vi "PicoScope5000aAdvancedTriggerSettingsV2.vi"(0 "error in":errorcluster, 1 "handle in":i16=16384, 3 "Trigger Conditions":T1 {"Digital Port 1" items=["Don't Care", "True", "False"]; "Digital Port 0" items=["Don't Care", "True", "False"]; "PWQ" items=["Don't Care", "True", "False"]; "Aux" items=["Don't Care", "True", "False"]; "Ext" items=["Don't Care", "True", "False"]; "Channel D" items=["Don't Care", "True", "False"]; "Channel C" items=["Don't Care", "True", "False"]; "Channel B" items=["Don't Care", "True", "False"]; "Channel A" items=["Don't Care", "True", "False"]; "Condition Logic" items=["AND", "OR", "XOR"]}, 4 "Trigger Delay":u32, 5 "Auto Trigger (us)":u64=1000000, 6 "Channel A Trigger Properties":T4={"thresholdUpper"=0, "thresholdUpperHysteresis"=0, "thresholdLower"=0, "thresholdLowerHysteresis"=0, "Threshold Mode"=0, "Direction"=2, "Available"=FALSE} {"Direction" items=["Above / Inside", "Below / Outside", "Rising / Enter", "Falling / Exit", "Rising or Falling / Enter or Exit", "Above Lower", "Below Lower", "Rising Lower", "Falling Lower", "Positive Runt", "Negative Runt"]; "Threshold Mode" items=["Level", "Window"]}, 7 "Channel D Trigger Properties":T4={"thresholdUpper"=0, "thresholdUpperHysteresis"=0, "thresholdLower"=0, "thresholdLowerHysteresis"=0, "Threshold Mode"=0, "Direction"=2, "Available"=FALSE} {"Direction" items=["Above / Inside", "Below / Outside", "Rising / Enter", "Falling / Exit", "Rising or Falling / Enter or Exit", "Above Lower", "Below Lower", "Rising Lower", "Falling Lower", "Positive Runt", "Negative Runt"]; "Threshold Mode" items=["Level", "Window"]}, 8 "Channel B Trigger Properties":T4={"thresholdUpper"=0, "thresholdUpperHysteresis"=0, "thresholdLower"=0, "thresholdLowerHysteresis"=0, "Threshold Mode"=0, "Direction"=2, "Available"=FALSE} {"Direction" items=["Above / Inside", "Below / Outside", "Rising / Enter", "Falling / Exit", "Rising or Falling / Enter or Exit", "Above Lower", "Below Lower", "Rising Lower", "Falling Lower", "Positive Runt", "Negative Runt"]; "Threshold Mode" items=["Level", "Window"]}, 10 "Digital Port  0":T3 {"Direction Channel 7" items=["Don't Care", "Low", "High", "Rising", "Falling"]; "Direction Channel 6" items=["Don't Care", "Low", "High", "Rising", "Falling"]; "Direction Channel 5" items=["Don't Care", "Low", "High", "Rising", "Falling"]; "Direction Channel 4" items=["Don't Care", "Low", "High", "Rising", "Falling"]; "Direction Channel 3" items=["Don't Care", "Low", "High", "Rising", "Falling"]; "Direction Channel 2" items=["Don't Care", "Low", "High", "Rising", "Falling"]; "Direction Channel 1" items=["Don't Care", "Low", "High", "Rising", "Falling"]; "Direction Channel 0" items=["Don't Care", "Low", "High", "Rising", "Falling"]}, 11 "Ext. Trigger Properties":T4={"thresholdUpper"=0, "thresholdUpperHysteresis"=0, "thresholdLower"=0, "thresholdLowerHysteresis"=0, "Threshold Mode"=0, "Direction"=2, "Available"=FALSE} {"Direction" items=["Above / Inside", "Below / Outside", "Rising / Enter", "Falling / Exit", "Rising or Falling / Enter or Exit", "Above Lower", "Below Lower", "Rising Lower", "Falling Lower", "Positive Runt", "Negative Runt"]; "Threshold Mode" items=["Level", "Window"]}, 12 "Digital Port  1":T2 {"Direction Channel 15" items=["Don't Care", "Low", "High", "Rising", "Falling"]; "Direction Channel 14" items=["Don't Care", "Low", "High", "Rising", "Falling"]; "Direction Channel 13" items=["Don't Care", "Low", "High", "Rising", "Falling"]; "Direction Channel 12" items=["Don't Care", "Low", "High", "Rising", "Falling"]; "Direction Channel 11" items=["Don't Care", "Low", "High", "Rising", "Falling"]; "Direction Channel 10" items=["Don't Care", "Low", "High", "Rising", "Falling"]; "Direction Channel 9" items=["Don't Care", "Low", "High", "Rising", "Falling"]; "Direction Channel 8" items=["Don't Care", "Low", "High", "Rising", "Falling"]}, 13 "Aux. Trigger Properties (DO NOT USE)":T4={"thresholdUpper"=0, "thresholdUpperHysteresis"=0, "thresholdLower"=0, "thresholdLowerHysteresis"=0, "Threshold Mode"=0, "Direction"=2, "Available"=FALSE} {"Direction" items=["Above / Inside", "Below / Outside", "Rising / Enter", "Falling / Exit", "Rising or Falling / Enter or Exit", "Above Lower", "Below Lower", "Rising Lower", "Falling Lower", "Positive Runt", "Negative Runt"]; "Threshold Mode" items=["Level", "Window"]}, 16 "Channel C Trigger Properties":T4={"thresholdUpper"=0, "thresholdUpperHysteresis"=0, "thresholdLower"=0, "thresholdLowerHysteresis"=0, "Threshold Mode"=0, "Direction"=2, "Available"=FALSE} {"Direction" items=["Above / Inside", "Below / Outside", "Rising / Enter", "Falling / Exit", "Rising or Falling / Enter or Exit", "Above Lower", "Below Lower", "Rising Lower", "Falling Lower", "Positive Runt", "Negative Runt"]; "Threshold Mode" items=["Level", "Window"]}, 18 "Pulse Width Qualifier Conditions":T6 {"Condition Logic" items=["AND", "OR", "XOR"]}, 19 "Pulse Width Qualifier Settings":T5={"Direction"=2, "Lower Limit"=0, "Upper Limit"=0, "Pulse Width Type"=0} {"Pulse Width Type" items=["None", "Less Than", "Greater Than", "In Range", "Out of Range"]; "Direction" items=["Rising"=2, "Falling"=3, "Rising Lower"=7, "Above"=0, "Below"=1, "Rising or Falling"=4, "Falling Lower"=8, "Below Lower"=6, "Above Lower"=5]}) -> (14 "error out":errorcluster, 15 "handle out":i16=16384)   [LabVIEW 2010]
doc: "This VI is an interface for the advanced trigger features of the oscilloscope (Using V2 functions now recommended)\nA simple trigger can be set using PicoScope5000aSettings.vi, in which case it is not necessary to use this VI."
uses:
  ps5000a.dll
panel:
  out "XOR Debug Array":u32[][](array[numeric])
  in  "SetTrigger Info Action XOR":bool=TRUE
  in  "SetTrigger Info Action OR":bool=TRUE
  # "For Condition Logic Suggested settings;\nFor AND, XOR logic-(parallel triggers)\nUse level-type triggers (Level or Inside/outside Window Triggers)\n\nFor OR logic- (single channel)\nUse edge types (e.g. rising, falling, entering window)"
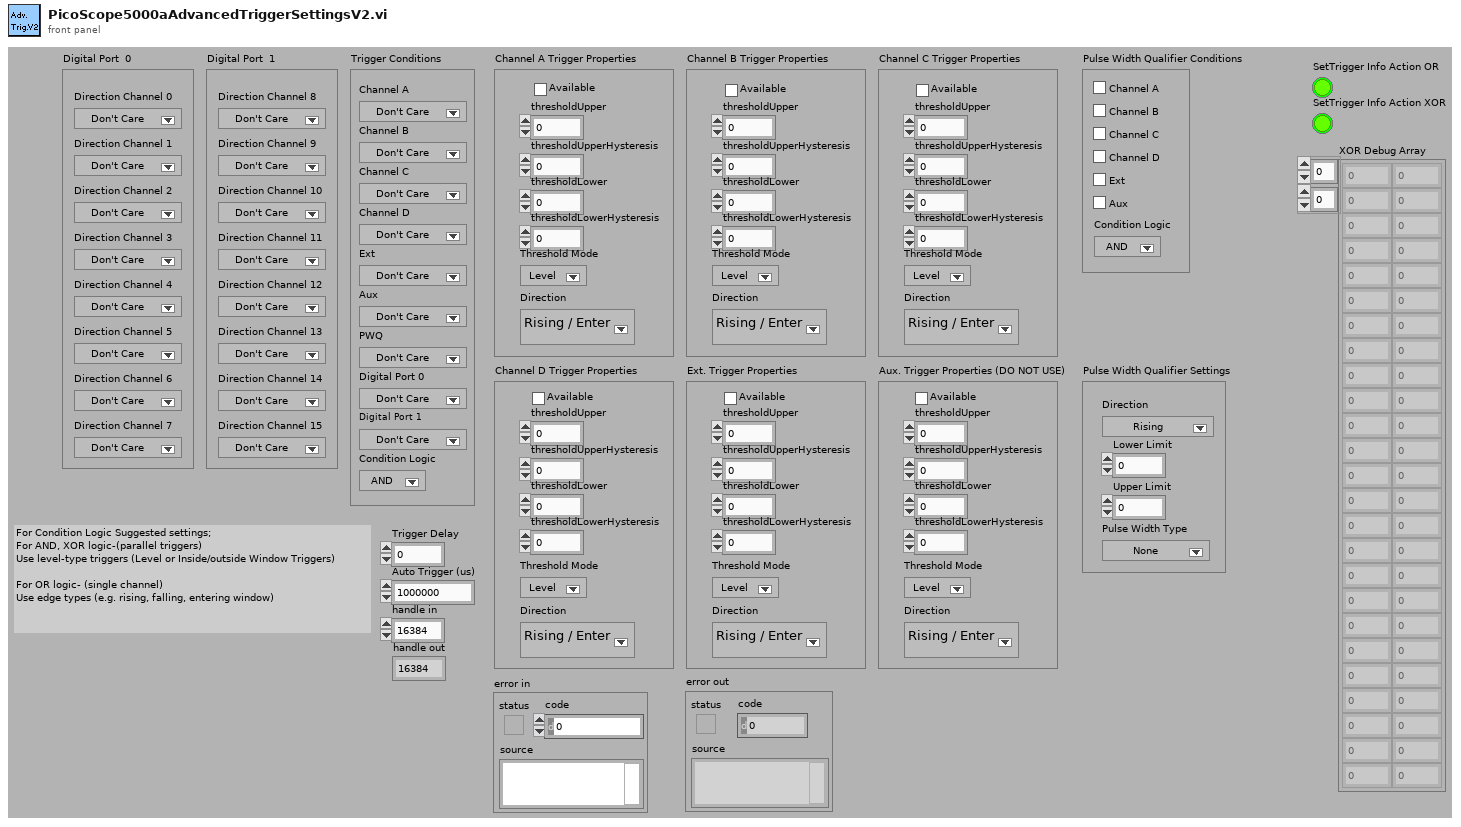
[diagram p1: front panel]
types:
  T1 = cluster{"Channel A":u16, "Channel B":u16, "Channel C":u16, "Channel D":u16, "Ext":u16, "Aux":u16, "PWQ":u16, "Digital Port 0":u16, "Digital Port 1":u16, "Condition Logic":u16}
  T2 = cluster{"Direction Channel 8":u16, "Direction Channel 9":u16, "Direction Channel 10":u16, "Direction Channel 11":u16, "Direction Channel 12":u16, "Direction Channel 13":u16, "Direction Channel 14":u16, "Direction Channel 15":u16}
  T3 = cluster{"Direction Channel 0":u16, "Direction Channel 1":u16, "Direction Channel 2":u16, "Direction Channel 3":u16, "Direction Channel 4":u16, "Direction Channel 5":u16, "Direction Channel 6":u16, "Direction Channel 7":u16}
  T4 = cluster{"thresholdUpper":i16, "thresholdUpperHysteresis":u16, "thresholdLower":i16, "thresholdLowerHysteresis":u16, "Threshold Mode":i32, "Direction":i32, "Available":bool}
  T5 = cluster{"Direction":u32, "Lower Limit":u32, "Upper Limit":u32, "Pulse Width Type":u32}
  T6 = cluster{"Channel A":bool, "Channel B":bool, "Channel C":bool, "Channel D":bool, "Aux":bool, "Condition Logic":u16, "Ext":bool}
  T7 = cluster{"thresholdUpper":i16, "thresholdUpperHysteresis":u16, "thresholdLower":i16, "thresholdLowerHysteresis":u16, "Threshold Mode":i32, "Direction":i32, "Available":bool}[]
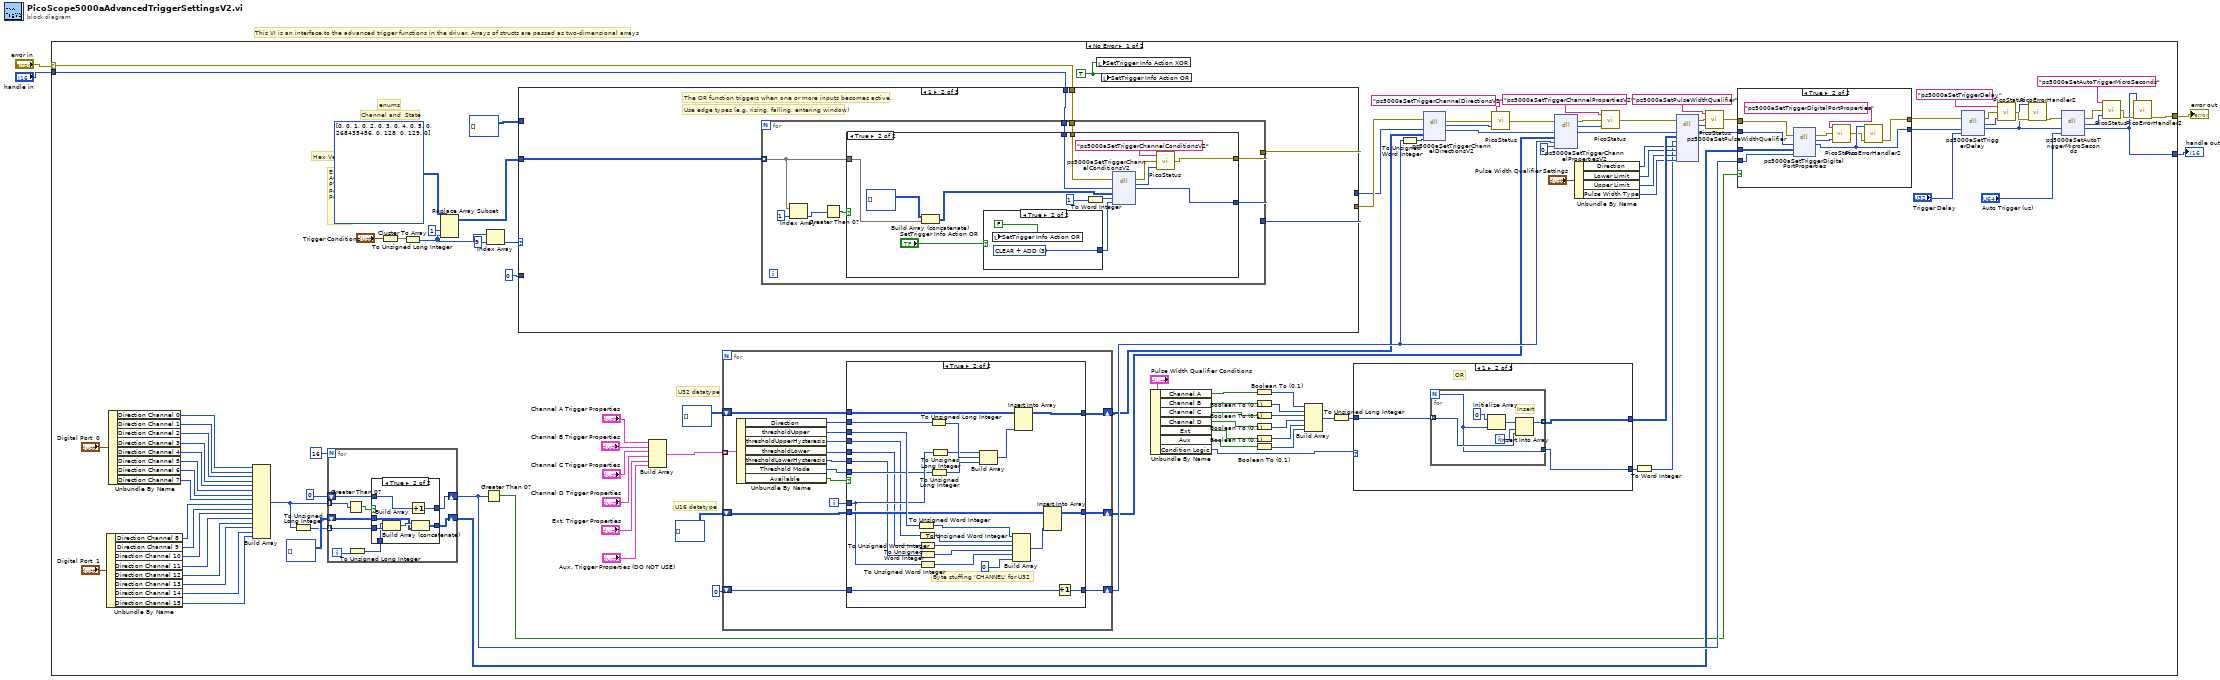
[diagram p0: block diagram]
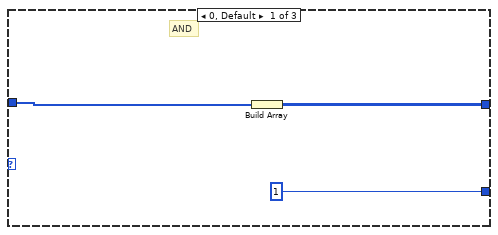
[diagram p4: hidden frame]
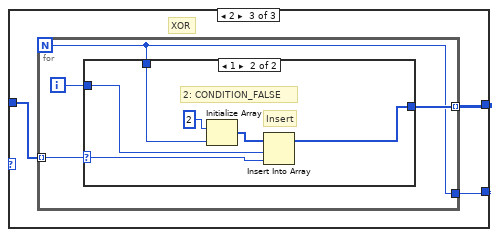
[diagram p5: hidden frame]
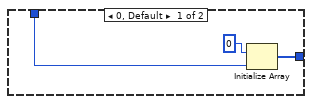
[diagram p6: hidden frame]
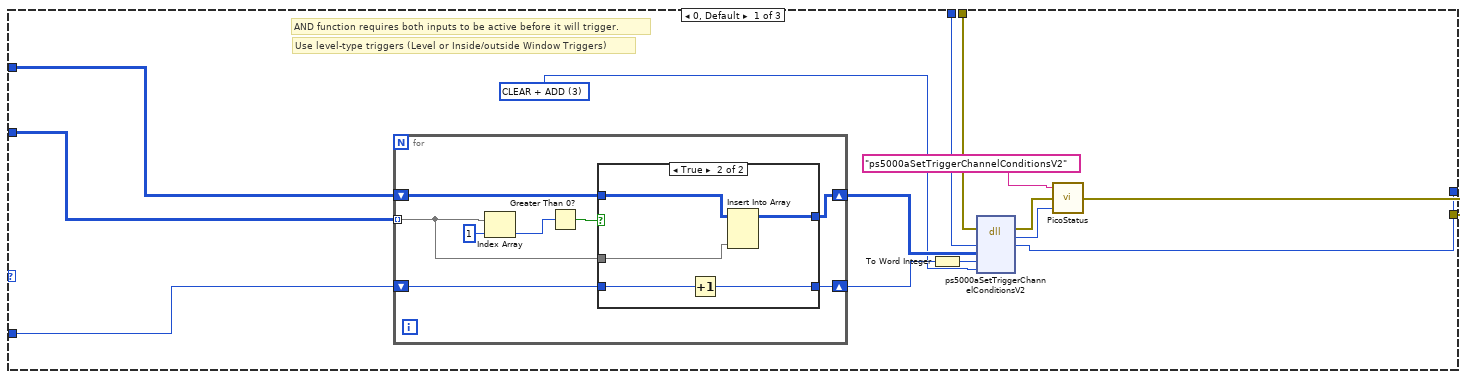
[diagram p8: hidden frame]
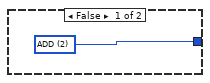
[diagram p11: hidden frame]
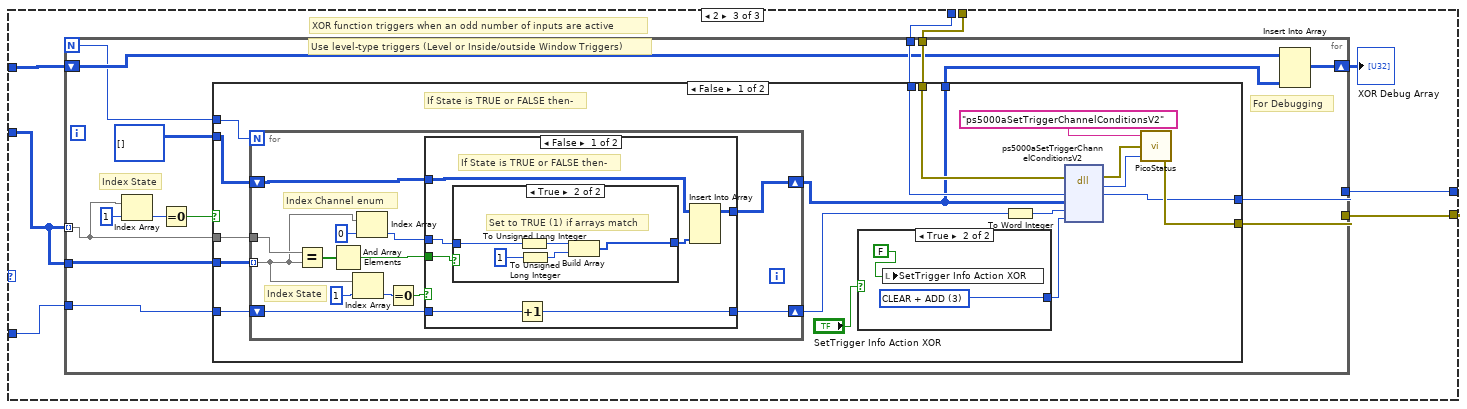
[diagram p12: hidden frame]
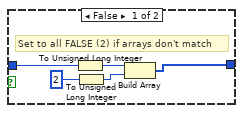
[diagram p13: hidden frame]
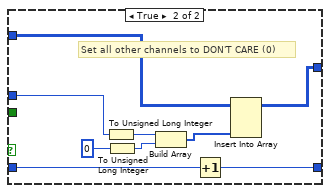
[diagram p14: hidden frame]
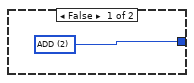
[diagram p15: hidden frame]
diagram:
  # "This VI is an interface to the advanced trigger functions in the driver. Arrays of structs are passed as two-dimensional arrays"
  n1 = case shown="No Error" "error in" {
    selector: "error in" -> [w46 w362]
    tunnel: "handle in" -> [w45 w363]
    tunnel: [w33 w363] -> w2
    tunnel: [w34 w362] -> w1
    frame No Error {
      w39 = TRUE ("Boolean")
      # "enums"
      # "Ext\nAux\nPWQ\nPort0\nPort1"
      # "Channel and  State"
      # "Hex Values"
      # "U16 datatype"
      # "U32 datatype"
      n2 = Unbundle By Name("Digital Port  1") -> ("Direction Channel 8"=w71:u16, "Direction Channel 9"=w70:u16, "Direction Channel 10"=w69:u16, "Direction Channel 11"=w68:u16, "Direction Channel 12"=w67:u16, "Direction Channel 13"=w66:u16, "Direction Channel 14"=w65:u16, "Direction Channel 15"=w64:u16)
      n3 = Unbundle By Name("Digital Port  0") -> ("Direction Channel 0"=w63:u16, "Direction Channel 1"=w80:u16, "Direction Channel 2"=w79:u16, "Direction Channel 3"=w78:u16, "Direction Channel 4"=w77:u16, "Direction Channel 5"=w76:u16, "Direction Channel 6"=w75:u16, "Direction Channel 7"=w74:u16)
      n4 = Build Array(w63, w80, w79, w78, w77, w76, w75, w74, w71, w70, w69, w68, w67, w66, w65, w64) -> (w52:u16[])
      n5 = To Unsigned Long Integer(number=w52) -> (unsigned 32bit integer=w53:u32[])
      n6 = for {
        N: 16 -> [_]
        tunnel: w53 -> [w134] mode=indexing
        shift-right: [w135] -> w57
        shift-left: i16 0 -> [w136]
        shift-right: [w132] -> w56
        shift-left: u32[][] [] -> [w133]
        tunnel: w52 -> [w130] mode=indexing
        i -> [w129]
        n7 = Greater Than 0?(x=w130) -> (x > 0?=w131:bool)
        n8 = To Unsigned Long Integer(number=w129) -> (unsigned 32bit integer=w128:u32)
        n9 = case shown="True" w131 {
          tunnel: w136 -> [w138 w145]
          tunnel: [w138 w142] -> w135
          tunnel: w134 -> [_ w144]
          tunnel: w128 -> [_ w143]
          tunnel: w133 -> [w137 w140]
          tunnel: [w137 w139] -> w132
          frame False {
          }
          frame True {
            n10 = Build Array(w143, w144) -> (w141:u32[])
            n11 = Increment(x=w145) -> (x+1=w142:i16)
            n12 = Build Array (concatenate)(w141, w140) -> (w139:u32[][])
          }
        }
      }
      n13 = Cluster To Array(cluster="Trigger Conditions") -> (array=w28:u16[])
      n14 = To Unsigned Long Integer(number=w28) -> (unsigned 32bit integer=w26:u32[])
      n15 = Replace Array Subset(array=u32[][] [[0, 0], [1, 0], [2, 0], [3, 0], [4, 0], [5, 0], [268435456, 0], [128, 0], [129, 0]], new element=w26, index (col)=1 ("disabled index (col)")) -> (w27:u32[][])  [unwired: 1 in]
      n16 = Greater Than 0?(x=w57) -> (x > 0?=w32:bool)
      n17 = Index Array(array=w26, index=9) -> (element=w24:u32)
      n18 = case shown="1" w24 {
        tunnel: u32[][] [] -> [w229 _ w280]
        tunnel: i16 0 -> [w228 _ w277]
        tunnel: w46 -> [w222 w249 w284]
        tunnel: w45 -> [w221 w248 w283]
        tunnel: [w218 w247 w282] -> w44
        tunnel: [w217 w246 w281] -> w43
        tunnel: w27 -> [w216 w245 w278]
        frame 0, Default {
          w219 = u32 3 items=["CLEAR + ADD"=3, "CLEAR"=1, "ADD"=2] ("Condition Action")
          # "AND function requires both inputs to be active before it will trigger."
          # "Use level-type triggers (Level or Inside/outside Window Triggers)"
          n19 = for {
            shift-right: [w236] -> w224
            shift-left: w228 -> [w235]
            shift-right: [w234] -> w220
            shift-left: w229 -> [w237]
            tunnel: w216 -> [w232] mode=indexing
            n20 = Index Array(array=w232, index=1) -> (element=w231:u32)
            n21 = Greater Than 0?(x=w231) -> (x > 0?=w233:bool)
            n22 = case shown="True" w233 {
              tunnel: w237 -> [w239 w244]
              tunnel: [w239 w243] -> w234
              tunnel: [w238 w242] -> w236
              tunnel: w235 -> [w238 w241]
              tunnel: w232 -> [_ w240]
              frame False {
              }
              frame True {
                n23 = Increment(x=w241) -> (x+1=w242:i16)
                n24 = Insert Into Array(array=w244, new element=w240) -> (w243:u32[][])  [unwired: 2 in]
              }
            }
          }
          n25 = To Word Integer(number=w224) -> (16bit integer=w227:i16)
          n26 = dll-call lib="ps5000a.dll" fn="ps5000aSetTriggerChannelConditionsV2" ("ps3000.dll:_ps3000_open_unit@0")(error in=w222, "handle"=w221, "conditions"=w220, "nConditions"=w227, "info"=w219) -> (error out=w226:errorcluster, "PICO_STATUS"=w225:u32, "handle"=w217:i16)  [unwired: 5 in, 1 out]
          n27 = call "PicoStatus.vi"("PICO STATUS"=w225, "error in"=w226, "source"="ps5000aSetTriggerChannelConditionsV2") -> ("error out"=w218:errorcluster)
        }
        frame 1 {
          # "Use edge types (e.g. rising, falling, entering window)"
          # "The OR function triggers when one or more inputs becomes active."
          n28 = for {
            tunnel: w249 -> [w257]
            tunnel: w248 -> [w256]
            tunnel: [w255] -> w247
            tunnel: [w254] -> w246
            tunnel: w245 -> [w252] mode=indexing
            n29 = Index Array(array=w252, index=1) -> (element=w251:u32)
            n30 = Greater Than 0?(x=w251) -> (x > 0?=w250:bool)
            n31 = case shown="True" w250 {
              tunnel: w257 -> [w258 w269]
              tunnel: w256 -> [w259 w268]
              tunnel: [w258 w266] -> w255
              tunnel: [w259 w265] -> w254
              tunnel: w252 -> [_ w260]
              frame False {
              }
              frame True {
                n32 = Build Array (concatenate)(u32[][] [], w260) -> (w262:u32[][])
                n33 = case shown="True" "SetTrigger Info Action OR" {
                  tunnel: [w274 w276] -> w267
                  frame False {
                    w274 = u32 2 items=["CLEAR"=1, "ADD"=2, "CLEAR + ADD"=3] ("Condition Action")
                  }
                  frame True {
                    w276 = u32 3 items=["CLEAR"=1, "ADD"=2, "CLEAR + ADD"=3] ("Condition Action")
                    n34 = local write "SetTrigger Info Action OR"(FALSE ("Boolean")) -> ()
                  }
                }
                n35 = To Word Integer(number=i16 1) -> (16bit integer=w273:i16)
                n36 = dll-call lib="ps5000a.dll" fn="ps5000aSetTriggerChannelConditionsV2" ("ps3000.dll:_ps3000_open_unit@0")(error in=w269, "handle"=w268, "conditions"=w262, "nConditions"=w273, "info"=w267) -> (error out=w272:errorcluster, "PICO_STATUS"=w271:u32, "handle"=w265:i16)  [unwired: 5 in, 1 out]
                n37 = call "PicoStatus.vi"("PICO STATUS"=w271, "error in"=w272, "source"="ps5000aSetTriggerChannelConditionsV2") -> ("error out"=w266:errorcluster)
              }
            }
          }
        }
        frame 2 {
          # "Use level-type triggers (Level or Inside/outside Window Triggers)"
          # "XOR function triggers when an odd number of inputs are active"
          n38 = for {
            N -> [w292]
            tunnel: w284 -> [w299]
            tunnel: w283 -> [w298]
            tunnel: [w297] -> w282
            tunnel: [w296] -> w281
            shift-right: [w294] -> w279
            shift-left: w280 -> [w295]
            tunnel: w278 -> [w286] mode=indexing
            tunnel: w278 -> [w289]
            tunnel: w277 -> [w290]
            # "Index State"
            # "For Debugging"
            n39 = Index Array(array=w286, index=1) -> (element=w287:u32)
            n40 = Equal To 0?(x=w287) -> (x = 0?=w285:bool)
            n41 = case shown="False" w285 {
              tunnel: w299 -> [w316 w359]
              tunnel: w298 -> [w315 w360]
              tunnel: [w314 w359] -> w297
              tunnel: [w313 w360] -> w296
              tunnel: [w311 w361] -> w293
              tunnel: w292 -> [w310 _]
              tunnel: u32[][] [] -> [w309 w361]
              tunnel: w290 -> [w308 _]
              tunnel: w289 -> [w307 _]
              tunnel: w286 -> [w306 _]
              frame False {
                # "If State is TRUE or FALSE then-"
                n42 = for {
                  N: w310 -> [_]
                  shift-right: [w328] -> w312
                  shift-left: w308 -> [w329]
                  shift-right: [w317] -> w311
                  shift-left: w309 -> [w318]
                  tunnel: w306 -> [w325]
                  tunnel: w307 -> [w321] mode=indexing
                  # "Index State"
                  # "Index Channel enum"
                  n43 = Equal?(x=w325, y=w321) -> (x = y?=w319:bool[])
                  n44 = And Array Elements(Boolean array=w319) -> (logical AND=w324:bool)
                  n45 = Index Array(array=w321, index=1) -> (element=w322:u32)
                  n46 = Index Array(array=w321, index=0) -> (element=w326:u32)
                  n47 = Equal To 0?(x=w322) -> (x = 0?=w320:bool)
                  n48 = case shown="False" w320 {
                    tunnel: w329 -> [w336 w347]
                    tunnel: [w335 w348] -> w328
                    tunnel: w326 -> [w334 w351]
                    tunnel: w324 -> [w333 _]
                    tunnel: w318 -> [w332 w350]
                    tunnel: [w330 w349] -> w317
                    frame False {
                      # "If State is TRUE or FALSE then-"
                      n49 = case shown="True" w333 {
                        tunnel: [w341 w346] -> w331
                        tunnel: w334 -> [w340 w345]
                        frame False {
                          # "Set to all FALSE (2) if arrays don't match"
                          n50 = To Unsigned Long Integer(number=w340) -> (unsigned 32bit integer=w338:u32)
                          n51 = To Unsigned Long Integer(number=u32 2) -> (unsigned 32bit integer=w339:u32)
                          n52 = Build Array(w338, w339) -> (w341:u32[])
                        }
                        frame True {
                          # "Set to TRUE (1) if arrays match"
                          n53 = To Unsigned Long Integer(number=w345) -> (unsigned 32bit integer=w343:u32)
                          n54 = To Unsigned Long Integer(number=u32 1) -> (unsigned 32bit integer=w344:u32)
                          n55 = Build Array(w343, w344) -> (w346:u32[])
                        }
                      }
                      n56 = Increment(x=w336) -> (x+1=w335:i16)
                      n57 = Insert Into Array(array=w332, new element=w331) -> (w330:u32[][])  [unwired: 2 in]
                    }
                    frame True {
                      # "Set all other channels to DON'T CARE (0)"
                      n58 = To Unsigned Long Integer(number=w351) -> (unsigned 32bit integer=w353:u32)
                      n59 = To Unsigned Long Integer(number=u32 0) -> (unsigned 32bit integer=w354:u32)
                      n60 = Build Array(w353, w354) -> (w355:u32[])
                      n61 = Increment(x=w347) -> (x+1=w348:i16)
                      n62 = Insert Into Array(array=w350, new element=w355) -> (w349:u32[][])  [unwired: 2 in]
                    }
                  }
                }
                n63 = case shown="True" "SetTrigger Info Action XOR" {
                  tunnel: [w356 w358] -> w300
                  frame False {
                    w356 = u32 2 items=["CLEAR + ADD"=3, "CLEAR"=1, "ADD"=2] ("Condition Action")
                  }
                  frame True {
                    w358 = u32 3 items=["CLEAR + ADD"=3, "CLEAR"=1, "ADD"=2] ("Condition Action")
                    n64 = local write "SetTrigger Info Action XOR"(FALSE ("Boolean")) -> ()
                  }
                }
                n65 = To Word Integer(number=w312) -> (16bit integer=w305:i16)
                n66 = dll-call lib="ps5000a.dll" fn="ps5000aSetTriggerChannelConditionsV2" ("ps3000.dll:_ps3000_open_unit@0")(error in=w316, "handle"=w315, "conditions"=w311, "nConditions"=w305, "info"=w300) -> (error out=w304:errorcluster, "PICO_STATUS"=w303:u32, "handle"=w313:i16)  [unwired: 5 in, 1 out]
                n67 = call "PicoStatus.vi"("PICO STATUS"=w303, "error in"=w304, "source"="ps5000aSetTriggerChannelConditionsV2") -> ("error out"=w314:errorcluster)
              }
              frame True {
              }
            }
            n68 = Insert Into Array(array=w295, new element=w293) -> (w294:u32[][])  [unwired: 2 in]
          }
          "XOR Debug Array" <- w279
        }
      }
      n69 = Build Array("Channel A Trigger Properties", "Channel B Trigger Properties", "Channel C Trigger Properties", "Channel D Trigger Properties", "Ext. Trigger Properties", "Aux. Trigger Properties (DO NOT USE)") -> (w111:T7)
      n70 = for {
        tunnel: w111 -> [w183] mode=indexing
        shift-right: [w180] -> w49
        shift-left: i16 0 -> [w179]
        shift-right: [w177] -> w22
        shift-left: u16[][] [] -> [w178]
        shift-right: [w176] -> w23
        shift-left: u32[][] [] -> [w175]
        i -> [w181]
        n71 = Unbundle By Name(w183) -> ("Direction"=w174:i32, "thresholdUpper"=w188:i16, "thresholdUpperHysteresis"=w187:u16, "thresholdLower"=w186:i16, "thresholdLowerHysteresis"=w185:u16, "Threshold Mode"=w184:i32, "Available"=w182:bool)
        n72 = case shown="True" w182 {
          tunnel: w188 -> [_ w215]
          tunnel: w187 -> [_ w195]
          tunnel: w186 -> [_ w194]
          tunnel: w185 -> [_ w193]
          tunnel: w184 -> [_ w203]
          tunnel: w181 -> [_ w205]
          tunnel: [w191 w213] -> w180
          tunnel: w179 -> [w191 w212]
          tunnel: [w190 w210] -> w177
          tunnel: w178 -> [w190 w209]
          tunnel: [w189 w208] -> w176
          tunnel: w175 -> [w189 w207]
          tunnel: w174 -> [_ w204]
          frame False {
          }
          frame True {
            # "Byte stuffing 'CHANNEL' for U32"
            n73 = To Unsigned Word Integer(number=w215) -> (unsigned 16bit integer=w197:u16)
            n74 = To Unsigned Word Integer(number=w195) -> (unsigned 16bit integer=w196:u16)
            n75 = To Unsigned Word Integer(number=w194) -> (unsigned 16bit integer=w192:u16)
            n76 = To Unsigned Word Integer(number=w193) -> (unsigned 16bit integer=w198:u16)
            n77 = To Unsigned Word Integer(number=w205) -> (unsigned 16bit integer=w199:u16)
            n78 = To Unsigned Long Integer(number=w204) -> (unsigned 32bit integer=w201:u32)
            n79 = To Unsigned Long Integer(number=w203) -> (unsigned 32bit integer=w202:u32)
            n80 = To Unsigned Long Integer(number=w205) -> (unsigned 32bit integer=w200:u32)
            n81 = Build Array(w200, w201, w202) -> (w206:u32[])
            n82 = Build Array(w197, w196, w192, w198, w199, u16 0 ("element")) -> (w211:u16[])
            n83 = Insert Into Array(array=w207, new element=w206) -> (w208:u32[][])  [unwired: 2 in]
            n84 = Insert Into Array(array=w209, new element=w211) -> (w210:u16[][])  [unwired: 2 in]
            n85 = Increment(x=w212) -> (x+1=w213:i16)
          }
        }
      }
      n86 = local write "SetTrigger Info Action XOR"(w39) -> ()
      n87 = local write "SetTrigger Info Action OR"(w39) -> ()
      n88 = Unbundle By Name("Pulse Width Qualifier Conditions") -> ("Channel A"=w14:bool, "Channel B"=w13:bool, "Channel C"=w12:bool, "Channel D"=w11:bool, "Ext"=w10:bool, "Aux"=w9:bool, "Condition Logic"=w7:u16)
      n89 = Boolean To (0,1)(Boolean=w14) -> (0, 1=w17:i16)
      n90 = Boolean To (0,1)(Boolean=w13) -> (0, 1=w18:i16)
      n91 = Boolean To (0,1)(Boolean=w12) -> (0, 1=w19:i16)
      n92 = Boolean To (0,1)(Boolean=w11) -> (0, 1=w20:i16)
      n93 = Boolean To (0,1)(Boolean=w10) -> (0, 1=w21:i16)
      n94 = Boolean To (0,1)(Boolean=w9) -> (0, 1=w16:i16)
      n95 = Build Array(w17, w18, w19, w20, w21, w16) -> (w15:i16[])
      n96 = To Unsigned Long Integer(number=w15) -> (unsigned 32bit integer=w8:u32[])
      n97 = case shown="1" w7 {
        tunnel: [w148 w151 w160] -> w109
        tunnel: [u32 1 w149 w159] -> w6
        tunnel: w8 -> [w146 w150 w158]
        frame 0, Default {
          # "AND"
          n98 = Build Array(w146) -> (w148:u32[][])
        }
        frame 1 {
          # "OR"
          n99 = for {
            N -> [w152]
            tunnel: w150 -> [w154] mode=indexing
            tunnel: [w153] -> w151 mode=indexing
            tunnel: [w152] -> w149
            i -> [w155]
            # "Insert"
            n100 = Initialize Array(u32 0 ("element"), w152) -> (w156:u32[])
            n101 = Insert Into Array(array=w156, index=w155, new element=w154) -> (w153:u32[])
          }
        }
        frame 2 {
          # "XOR"
          n102 = for {
            N -> [w161]
            tunnel: w158 -> [w164] mode=indexing
            tunnel: [w162] -> w160 mode=indexing
            tunnel: [w161] -> w159
            i -> [w163]
            n103 = case shown="1" w164 {
              selector: w164 -> [_ w170]
              tunnel: [w166 w171] -> w162
              tunnel: w163 -> [_ w169]
              tunnel: w161 -> [w165 w168]
              frame 0, Default {
                n104 = Initialize Array(u32 0 ("element"), w165) -> (w166:u32[])
              }
              frame 1 {
                # "2: CONDITION_FALSE"
                # "Insert"
                n105 = Initialize Array(u32 2 ("element"), w168) -> (w172:u32[])
                n106 = Insert Into Array(array=w172, index=w169, new element=w170) -> (w171:u32[])
              }
            }
          }
        }
      }
      n107 = To Unsigned Word Integer(number=w49) -> (unsigned 16bit integer=w50:u16)
      n108 = dll-call lib="ps5000a.dll" fn="ps5000aSetTriggerChannelDirectionsV2" ("ps3000.dll:_ps3000_open_unit@0")(error in=w44, "handle"=w43, "directions"=w23, "nDirections"=w50) -> (error out=w97:errorcluster, "PICO_STATUS"=w98:u32, "handle"=w114:i16)  [unwired: 4 in, 1 out]
      n109 = call "PicoStatus.vi"("PICO STATUS"=w98, "error in"=w97, "source"="ps5000aSetTriggerChannelDirectionsV2") -> ("error out"=w89:errorcluster)
      n110 = dll-call lib="ps5000a.dll" fn="ps5000aSetTriggerChannelPropertiesV2" ("ps3000.dll:_ps3000_open_unit@0")(error in=w89, "handle"=w114, "channelProperties"=w22, "nChannelProperties"=w49, "auxOutputEnable"=i16 0) -> (error out=w95:errorcluster, "PICO_STATUS"=w96:u32, "handle"=w113:i16)  [unwired: 5 in, 1 out]
      n111 = Unbundle By Name("Pulse Width Qualifier Settings") -> ("Direction"=w107:u32, "Lower Limit"=w106:u32, "Upper Limit"=w105:u32, "Pulse Width Type"=w104:u32)
      n112 = call "PicoStatus.vi"("PICO STATUS"=w96, "error in"=w95, "source"="ps5000aSetTriggerChannelPropertiesV2") -> ("error out"=w88:errorcluster)
      n113 = To Word Integer(number=w6) -> (16bit integer=w5:i16)
      n114 = dll-call lib="ps5000a.dll" fn="ps5000aSetPulseWidthQualifier" ("ps3000.dll:_ps3000_open_unit@0")(error in=w88, "handle"=w113, "conditions"=w109, "nConditions"=w5, "direction"=w107, "lower"=w106, "upper"=w105, "type"=w104) -> (error out=w93:errorcluster, "PICO_STATUS"=w94:u32, "handle"=w59:i16)  [unwired: 8 in, 1 out]
      n115 = call "PicoStatus.vi"("PICO STATUS"=w94, "error in"=w93, "source"="ps5000aSetPulseWidthQualifier") -> ("error out"=w58:errorcluster)
      n116 = case shown="True" w32 {
        tunnel: w59 -> [w116 w124]
        tunnel: w58 -> [w117 w123]
        tunnel: w57 -> [_ w122]
        tunnel: w56 -> [_ w121]
        tunnel: [w117 w118] -> w55
        tunnel: [w116 w120] -> w54
        frame False {
        }
        frame True {
          n117 = dll-call lib="ps5000a.dll" fn="ps5000aSetTriggerDigitalPortProperties"(error in=w123, "handle"=w124, "digitalDirections"=w121, "nDigitalDirections"=w122) -> (error out=w126:errorcluster, "PICO_STATUS"=w125:u32, "handle"=w120:i16)  [unwired: 4 in, 1 out]
          n118 = call "PicoStatus.vi"("PICO STATUS"=w125, "error in"=w126, "source"="ps5000aSetTriggerDigitalPortProperties") -> ("error out"=w119:errorcluster)
          n119 = call "PicoErrorHandler2.vi"("error in (no error)"=w119, "handle In"=w120) -> ("error out"=w118:errorcluster)  [unwired: 9 in]
        }
      }
      n120 = dll-call lib="ps5000a.dll" fn="ps5000aSetTriggerDelay" ("ps3000.dll:_ps3000_open_unit@0")(error in=w55, "handle"=w54, "delay"="Trigger Delay") -> (error out=w91:errorcluster, "PICO_STATUS"=w92:u32, "handle"=w41:i16)  [unwired: 3 in, 1 out]
      n121 = call "PicoStatus.vi"("PICO STATUS"=w92, "error in"=w91, "source"="ps5000aSetTriggerDelay") -> ("error out"=w90:errorcluster)
      n122 = call "PicoErrorHandler2.vi"("error in (no error)"=w90, "handle In"=w41) -> ("error out"=w42:errorcluster)  [unwired: 9 in]
      n123 = dll-call lib="ps5000a.dll" fn="ps5000aSetAutoTriggerMicroSeconds" ("ps3000.dll:_ps3000_open_unit@0")(error in=w42, "handle"=w41, "autoTriggerMicroseconds"="Auto Trigger (us)") -> (error out=w37:errorcluster, "PICO_STATUS"=w36:u32, "handle"=w33:i16)  [unwired: 3 in, 1 out]
      n124 = call "PicoStatus.vi"("PICO STATUS"=w36, "error in"=w37, "source"="ps5000aSetAutoTriggerMicroSeconds") -> ("error out"=w38:errorcluster)
      n125 = call "PicoErrorHandler2.vi"("error in (no error)"=w38, "handle In"=w33) -> ("error out"=w34:errorcluster)  [unwired: 9 in]
    }
    frame Error {
    }
  }
  "handle out" <- w2
  "error out" <- w1
